vi "Write Active Dot.vi"(8 "error in (no error)":errorcluster, 10 "Active Dot":refnum<class "Dot Settings.lvclass">, 11 "Setting Database in":refnum<class "Setting Database.lvclass">) -> (0 "error out":errorcluster, 3 "Setting Database out":refnum<class "Setting Database.lvclass">)   [LabVIEW 2019, in "Setting Database.lvclass"]
uses:
  Setting Database.lvclass
  Dot Settings/Dot Settings.lvclass
  ObjectSettings/Accessors/Read Enabled.vi
  ObjectSettings/Accessors/Write Enabled.vi
  C:/Users/Albro/Documents/GitHub/AFM-Lithography/lvsrc/Classes/Settings/ObjectSettings/ObjectSettings.lvclass
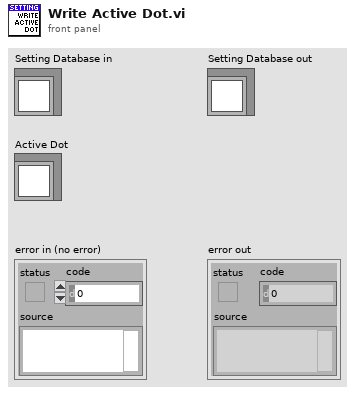
[diagram p1: front panel]
types:
  T1 = cluster{"Path":string, "Funnel":string, "Rectangle":string, "Dot":string}
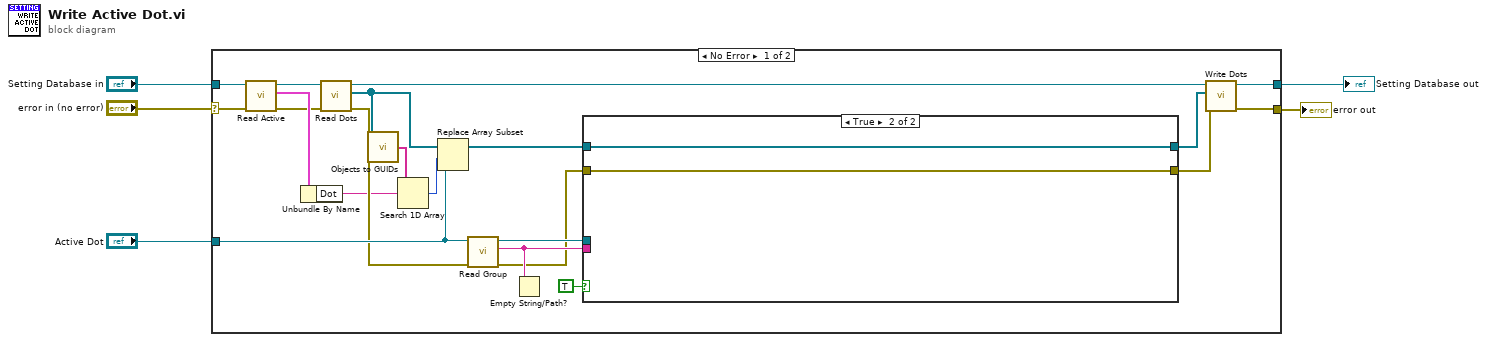
[diagram p0: block diagram]
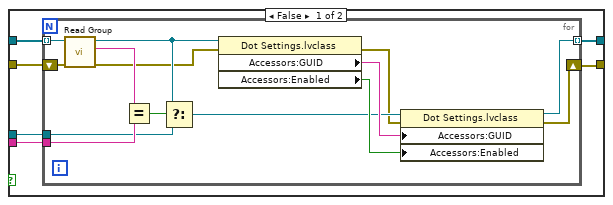
[diagram p2: hidden frame]
diagram:
  n1 = case shown="No Error" "error in (no error)" {
    selector: "error in (no error)" -> [w26 w50]
    tunnel: [w11 w50] -> w1
    tunnel: [w12 w49] -> w2
    tunnel: "Setting Database in" -> [w25 w49]
    tunnel: "Active Dot" -> [w23 _]
    frame No Error {
      n2 = call "Read Active.vi"("error in (no error)"=w26, "Setting Database in"=w25) -> ("error out"=w16:errorcluster, "Active"=w24:T1, "Setting Database out"=w18:refnum<class "Setting Database.lvclass">)  [unwired: 7 in]
      n3 = Unbundle By Name(w24) -> ("Dot"=w7:string)
      n4 = call "Read Dots.vi"("error in (no error)"=w16, "Setting Database in"=w18) -> ("error out"=w17:errorcluster, "Dots"=w9:refnum<class "Dot Settings.lvclass">[], "Setting Database out"=w15:refnum<class "Setting Database.lvclass">)  [unwired: 7 in]
      n5 = call "Objects to GUIDs.vi"("Objects"=w9) -> ("GUIDs"=w8:string[])  [unwired: 3 in, 1 out]
      n6 = Search 1D Array(1D array=w8, element=w7) -> (index of element=w6:i32)  [unwired: 1 in]
      n7 = Replace Array Subset(array=w9, new element=w23, index=w6) -> (w22:refnum<class "Dot Settings.lvclass">[])
      n8 = call-dynamic "Read Group.vi"("error in (no error)"=w17, "ObjectSettings in"=w23) -> ("error out"=w19:errorcluster, "Group"=w21:string, "ObjectSettings out"=w20:refnum<class "Dot Settings.lvclass">)  [unwired: 7 in]
      n9 = Empty String/Path?(string/path=w21) -> ()  [unwired: 1 out]
      n10 = case shown="True" TRUE {
        tunnel: w22 -> [w31 w48]
        tunnel: [w29 w48] -> w14
        tunnel: w21 -> [w32 _]
        tunnel: w20 -> [w30 _]
        tunnel: w19 -> [w28 w47]
        tunnel: [w27 w47] -> w13
        frame False {
          n11 = for {
            tunnel: w32 -> [w44]
            tunnel: w31 -> [w46] mode=indexing
            tunnel: w30 -> [w43]
            tunnel: [w41] -> w29 mode=indexing
            shift-right: [w33] -> w27
            shift-left: w28 -> [w34]
            n12 = call-dynamic "Read Group.vi"("error in (no error)"=w34, "ObjectSettings in"=w46) -> ("error out"=w35:errorcluster, "Group"=w45:string, "ObjectSettings out"=w42:refnum<class "Dot Settings.lvclass">)  [unwired: 7 in]
            n13 = Equal?(x=w45, y=w44) -> (x = y?=w37:bool)
            n14 = Select(t=w42, s=w37, f=w43) -> (s? t:f=w38:refnum<class "Dot Settings.lvclass">)
            n15 = property class="Dot Settings.lvclass"(reference=w42, error in=w35) -> (error out=w36:errorcluster, "Accessors:GUID"=w40:string, "Accessors:Enabled"=w39:bool)  [unwired: 1 out]
            n16 = property class="Dot Settings.lvclass"(reference=w38, error in=w36, "Accessors:GUID"=w40, "Accessors:Enabled"=w39) -> (reference out=w41:refnum<class "Dot Settings.lvclass">, error out=w33:errorcluster)
          }
        }
        frame True {
        }
      }
      n17 = call "Write Dots.vi"("error in (no error)"=w13, "Dots"=w14, "Setting Database in"=w15) -> ("error out"=w11:errorcluster, "Setting Database out"=w12:refnum<class "Setting Database.lvclass">)  [unwired: 7 in]
    }
    frame Error {
    }
  }
  "error out" <- w1
  "Setting Database out" <- w2
